vi "termometro.vi"() -> ()   [LabVIEW 2026]
panel:
  out "?":string
  out "?":string
  out ">10 C":bool
  out "<80 C":bool
  out "Celcius(C)":dbl(slide) scale=135.0..150.0
  out "kelvin(K)":dbl(slide) scale=-150.0..800.0
  out "farenheith (F)":dbl(slide) scale=-150.0..500.0
  in  "stop":bool
  in  "Slide":dbl(slide) scale=-100.0..200.0
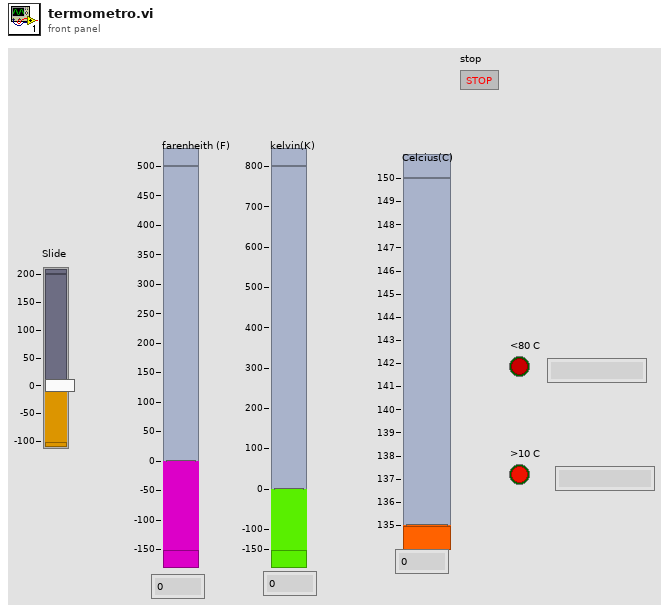
[diagram p1: front panel]
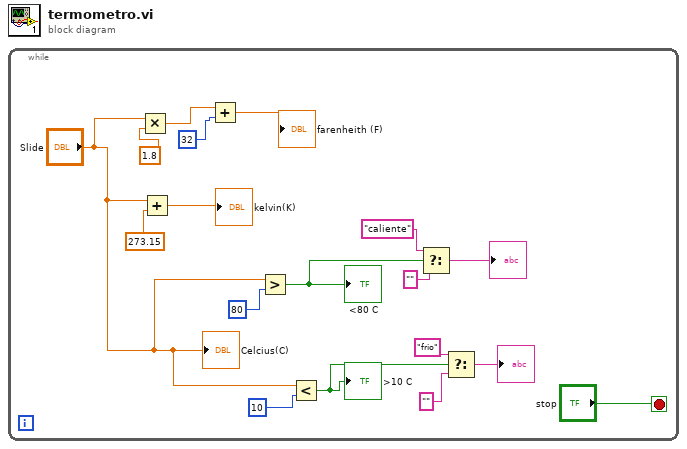
[diagram p0: block diagram]
diagram:
  n1 = while {
    stop <- "stop" stop-if-true
    n2 = Multiply(x="Slide", y=1.8) -> (x*y=w15:dbl)
    n3 = Add(x="Slide", y=273.15) -> (x+y=→"kelvin(K)":dbl)
    n4 = Add(x=w15, y=32) -> (x+y=→"farenheith (F)":dbl)
    n5 = Greater?(x="Slide", y=80) -> (0:w8:bool)
    "<80 C" <- w8
    n6 = Less?(x="Slide", y=10) -> (x < y?=w3:bool)
    ">10 C" <- w3
    n7 = Select(t="caliente", s=w8, f="") -> (s? t:f=→"?":string)
    n8 = Select(t="frio", s=w3, f="") -> (s? t:f=→"?":string)
    "Celcius(C)" <- "Slide"
  }
